vi "1.Create_Profile.vi"(8 "error out":errorcluster {"code" format="%.0x"}) -> (0 "error out":errorcluster {"code" format="%.0x"})   [LabVIEW 2021]
uses:
  test_type.ctl
  create profile state machine.ctl
panel:
  out "DCW":string[](array[string])
  out "output array":string[](array[string])
  out "IR":string[](array[string])
  out "Boolean":bool=TRUE
  out "Numeric":i32
  in  "Back Button":bool
  out "PROFILE TYPE 2":T1
  in  "String Indicator":string
  in  "Save Button":bool
  in  "Tab Control":enum32{"NA", "DCW", "ACW", "IR"}(tab)
  in  "DCW HI SET current value(mA)":sgl=11.0 min=0.001 max=11 format="%.3f"
  in  "DCW LO SET current value(mA)":sgl min=0 max=10.9 format="%.3f"
  in  "DCW Test Time(S)":sgl=0.5 min=0.5 max=999.9 format="%.1f"
  in  "DCW voltage(kV)":sgl=0.1 min=0.1 max=6.1 format="%.3f"
  in  "DCW Ramp Time":sgl=0.1 min=0.1 max=999.9 format="%.1f"
  in  "IR LO SET resistance value(M Ohm)":u16=2 min=1 max=9999
  in  "IR HI SET resistance value(M Ohm)":u16=9999 min=2 max=9999
  in  "IR Test Time(S)":sgl=1.0 min=1 max=999.9 format="%.1f"
  in  "Ramp Time":sgl=0.1 min=0.1 max=999.9 format="%.1f"
  in  "IR voltage(kV)":sgl=0.1 min=0.0499 max=1.0001 step=0.05 format="%.2f"
  in  "ACW Test Frequency(Hz)":u8(ring)=1 items=["50", "60"]
  in  "ACW Test Time(S)":sgl=0.5 min=0.5 max=999.9 format="%.1f"
  in  "ACW HI SET current value(mA)":sgl=42.0 min=0.001 max=42 format="%.3f"
  in  "ACW LO SET current value(mA)":sgl min=0 max=41.9 format="%.3f"
  in  "ACW voltage(kV)":sgl=0.1 min=0.1 max=5 format="%.3f"
  in  "ACW Ramp Time":sgl=0.1 min=0.1 max=999.9 format="%.1f"
  in  "PROFILE TYPE":T1
  # "CREATE PROFILE"
  # "PROFILE NAME"
  # "MODE"
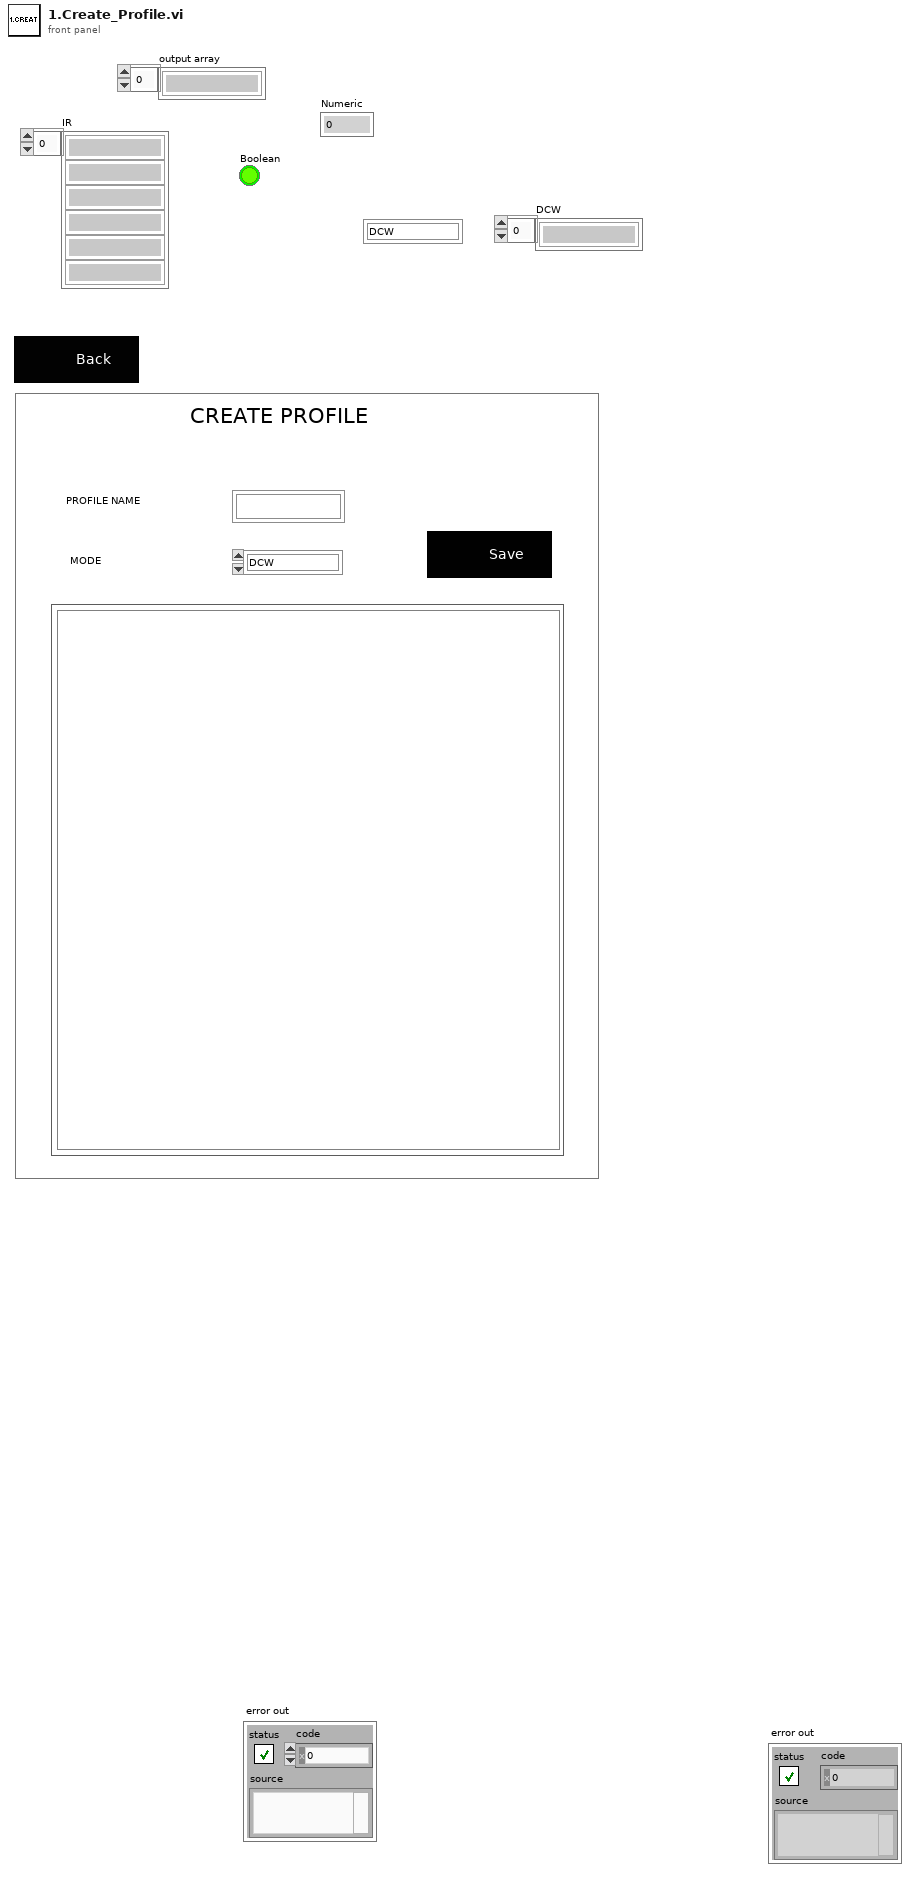
[diagram p1: front panel]
types:
  T1 = typedef "test_type.ctl" = enum16{"DCW", "ACW", "IR"}
  T2 = typedef "create profile state machine.ctl" = enum16{"Selection", "Compare name"}
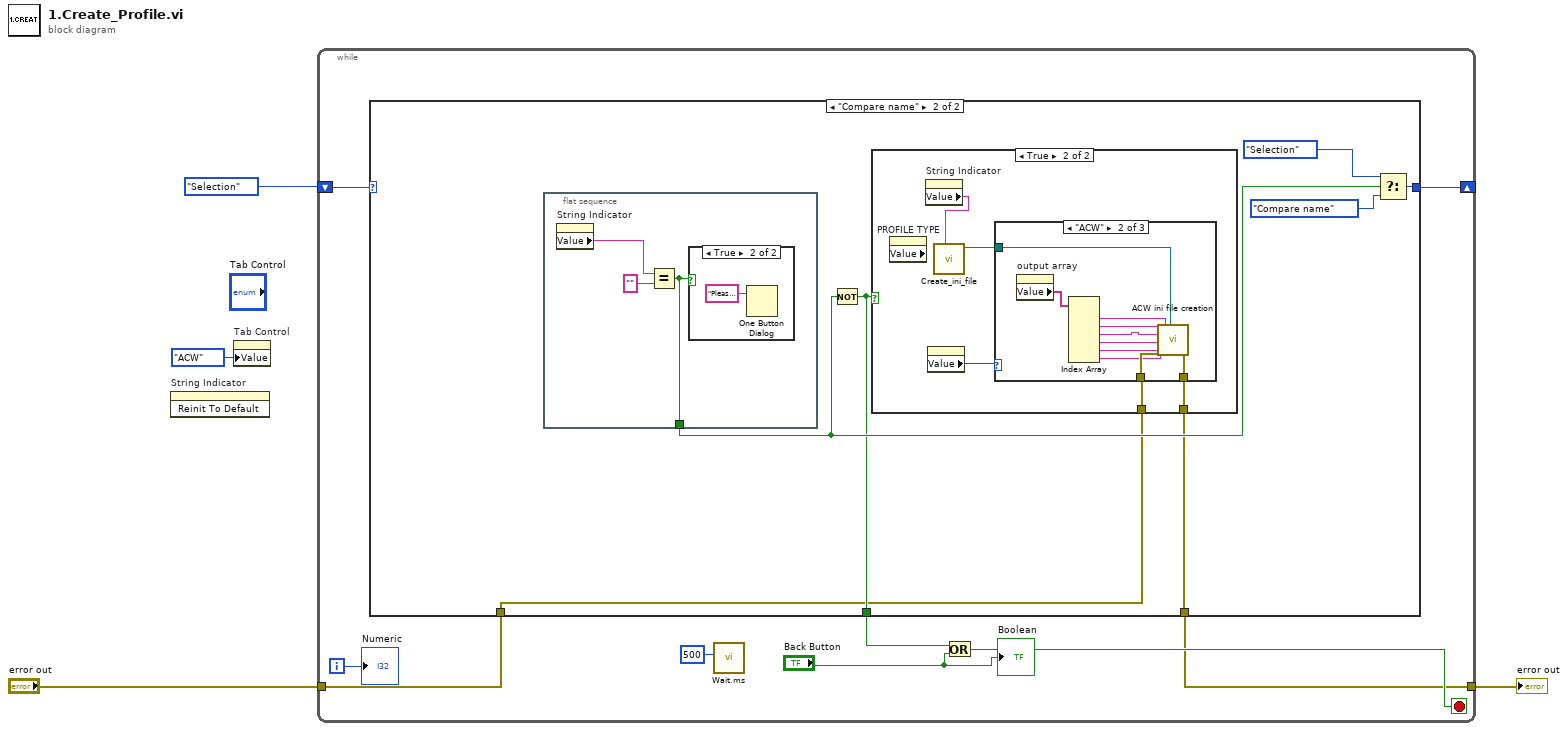
[diagram p0: block diagram]
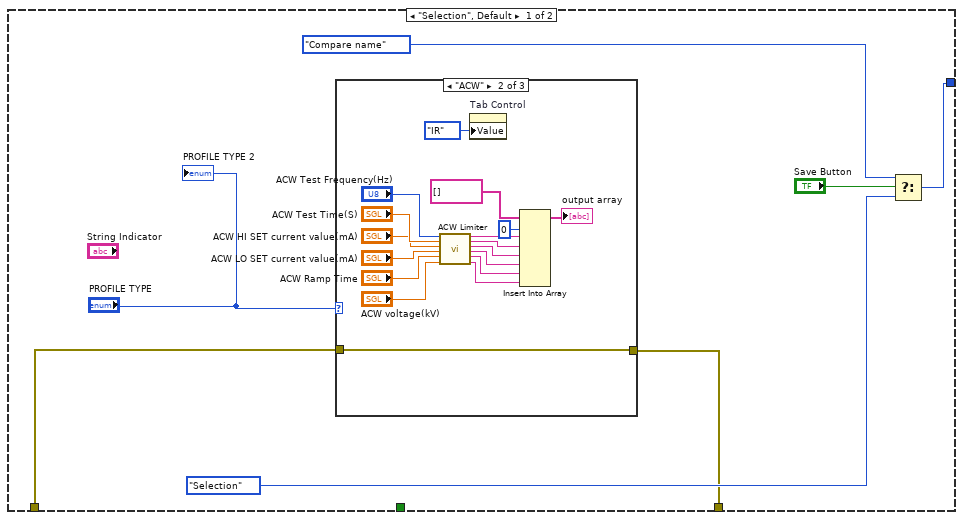
[diagram p2: hidden frame]
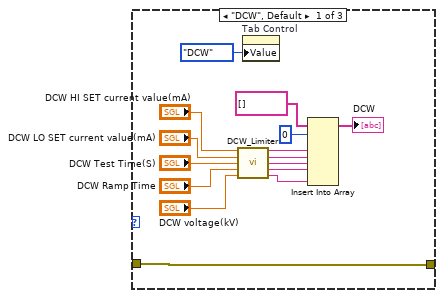
[diagram p3: hidden frame]
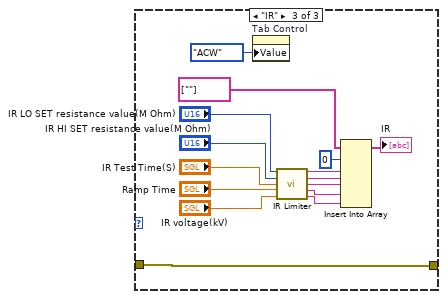
[diagram p4: hidden frame]
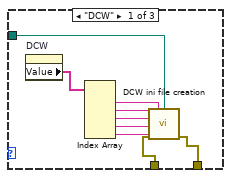
[diagram p6: hidden frame]
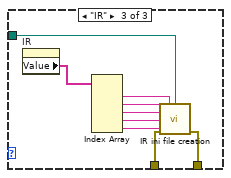
[diagram p7: hidden frame]
diagram:
  n1 = invoke on="String Indicator" class="Str" method="Reinit To Default"() -> ()  [unwired: 3 in, 3 out]
  n2 = property on="Tab Control" class="TabCtl (strict)"("Value"=enum32{"NA", "DCW", "ACW", "IR"}."ACW" ("Tab Control")) -> ()  [unwired: 2 in, 2 out]
  n3 = while {
    shift-right: [w12] -> _
    shift-left: create_profile_state_machine."Selection" -> [w13]
    tunnel: "error out" -> [w5]
    tunnel: [w6] -> w1
    i -> [w8]
    stop <- w9 stop-if-true
    n4 = case shown="\"Compare name\"" w13 {
      tunnel: [w20 w73] -> w12
      tunnel: w5 -> [w16 w68]
      tunnel: [_ w70] -> w10
      tunnel: [w14 w69] -> w6
      frame "Selection", Default {
        n5 = case shown="\"ACW\"" "PROFILE TYPE" {
          tunnel: w16 -> [w34 w51 w66]
          tunnel: [w34 w51 w66] -> w14
          frame "DCW", Default {
            n6 = call "DCW_Limiter.vi"("DCW HI SET current value(mA)"="DCW HI SET current value(mA)", "DCW LO SET current value(mA)"="DCW LO SET current value(mA)", "DCW Test Time(S)"="DCW Test Time(S)", "Ramp Time"="DCW Ramp Time", "DCW voltage(kV)"="DCW voltage(kV)") -> ("DCW voltage(kV)"=w33:string, "Ramp Time"=w32:string, "DCW LO SET current value(mA)"=w31:string, "DCW HI SET current value(mA)"=w30:string, "DCW Test Time(S)"=w29:string)  [unwired: 6 in]
            n7 = property on="Tab Control" class="TabCtl (strict)"("Value"=enum32{"NA", "DCW", "ACW", "IR"}."DCW" ("Tab Control")) -> ()  [unwired: 2 in, 2 out]
            n8 = Insert Into Array(array=string[] [], index=0, new element #1=w33, new element #2=w32, new element #3=w31, new element #4=w30, new element #5=w29) -> (→"DCW":string[])
          }
          frame "ACW" {
            n9 = call "ACW Limiter.vi"("ACW Test Frequency(Hz)"="ACW Test Frequency(Hz)", "ACW Test Time(S)"="ACW Test Time(S)", "ACW HI SET current value(mA)"="ACW HI SET current value(mA)", "ACW LO SET current value(mA)"="ACW LO SET current value(mA)", "Ramp Time"="ACW Ramp Time", "ACW voltage(kV)"="ACW voltage(kV)") -> ("ACW voltage(kV)"=w50:string, "Ramp Time"=w49:string, "ACW LO SET current value(mA)"=w48:string, "ACW HI SET current value(mA)"=w47:string, "ACW Test Time(S)"=w46:string, "ACW Test Frequency(Hz)"=w45:string)  [unwired: 8 in]
            n10 = property on="Tab Control" class="TabCtl (strict)"("Value"=enum32{"NA", "DCW", "ACW", "IR"}."IR" ("Tab Control")) -> ()  [unwired: 2 in, 2 out]
            n11 = Insert Into Array(array=string[] [], index=0, new element #1=w50, new element #2=w49, new element #3=w48, new element #4=w47, new element #5=w46, new element #6=w45) -> (→"output array":string[])
          }
          frame "IR" {
            n12 = property on="Tab Control" class="TabCtl (strict)"("Value"=enum32{"NA", "DCW", "ACW", "IR"}."ACW" ("Tab Control")) -> ()  [unwired: 2 in, 2 out]
            n13 = call "IR Limiter.vi"("IR LO SET resistance value(M£[)"="IR LO SET resistance value(M Ohm)", "IR HI SET resistance value(M£[)"="IR HI SET resistance value(M Ohm)", "IR Test Time(S)"="IR Test Time(S)", "Ramp Time"="Ramp Time", "IR voltage(kV)"="IR voltage(kV)") -> ("IR voltage(kV)"=w65:string, "IR Test Time(S)"=w64:string, "IR LO SET"=w63:string, "IR HI SET"=w62:string, "Ramp Time"=w61:string)  [unwired: 6 in]
            n14 = Insert Into Array(array=string[] [""], index=0, new element #1=w65, new element #2=w64, new element #3=w63, new element #4=w62, new element #5=w61) -> (→"IR":string[])
          }
        }
        n15 = Select(t=create_profile_state_machine."Compare name", s="Save Button", f=create_profile_state_machine."Selection") -> (s? t:f=w20:T2)
        "PROFILE TYPE 2" <- "PROFILE TYPE"
      }
      frame "Compare name" {
        n16 = flat-sequence {
          tunnel: [w110] -> w71
          frame #0 {
            n17 = property on="String Indicator" class="Str"() -> ("Value"=w109:string)  [unwired: 2 in, 2 out]
            n18 = Equal?(x=w109, y="") -> (x = y?=w110:bool)
            n19 = case shown="True" w110 {
              frame False {
              }
              frame True {
                n20 = One Button Dialog(message="Please enter the Profile Name") -> ()  [unwired: 1 in, 1 out]
              }
            }
          }
        }
        n21 = Not(x=w71) -> (.not. x?=w70:bool)
        n22 = case shown="True" w70 {
          tunnel: [w75 w77] -> w69
          tunnel: w68 -> [w75 w76]
          frame False {
          }
          frame True {
            n23 = property on="PROFILE TYPE" class="Enum (strict)" props=["Value"]() -> ()  [unwired: 2 in, 3 out]
            n24 = property on="String Indicator" class="Str"() -> ("Value"=w79:string)  [unwired: 2 in, 2 out]
            n25 = property on="PROFILE TYPE 2" class="Enum (strict)"() -> ("Value"=w78:T1)  [unwired: 2 in, 2 out]
            n26 = call "Create_ini_file.vi"("Name"=w79) -> ("path"=w80:path)  [unwired: 9 in, 1 out]
            n27 = case shown="\"ACW\"" w78 {
              tunnel: w80 -> [w89 w95 w108]
              tunnel: [w88 w99 w107] -> w77
              tunnel: w76 -> [w87 w98 w106]
              frame "DCW" {
                n28 = property on="DCW" class="Arr (strict)"() -> ("Value"=w86:string[])  [unwired: 2 in, 2 out]
                n29 = Index Array(array=w86) -> (element #1=w85:string, element #2=w84:string, element #3=w83:string, element #4=w82:string, element #5=w81:string)  [unwired: 5 in]
                n30 = call "DCW ini file creation.vi"("Ramp Time"=w84, "DCW voltage(kV)"=w85, "configuration file path"=w89, "DCW LO SET current value(mA)"=w83, "DCW HI SET current value(mA)"=w82, "DCW Test Time(S)"=w81, "error in (no error) 2"=w87) -> ("error in (no error) 3"=w88:errorcluster)  [unwired: 8 in]
              }
              frame "ACW" {
                n31 = property on="output array" class="Arr (strict)"() -> ("Value"=w97:string[])  [unwired: 2 in, 2 out]
                n32 = Index Array(array=w97) -> (element #1=w96:string, element #2=w94:string, element #3=w93:string, element #4=w92:string, element #5=w90:string, element #6=w91:string)  [unwired: 6 in]
                n33 = call "ACW ini file creation.vi"("Ramp Time"=w94, "ACW LO SET current value(mA)"=w93, "ACW HI SET current value(mA)"=w92, "ACW Test Time(S)"=w90, "ACW Test Frequency(Hz)"=w91, "error in (no error) 2"=w98, "ACW voltage(kV)"=w96, "configuration file path"=w95) -> ("error in (no error) 3"=w99:errorcluster)  [unwired: 11 in]
              }
              frame "IR" {
                n34 = property on="IR" class="Arr (strict)"() -> ("Value"=w105:string[])  [unwired: 2 in, 2 out]
                n35 = Index Array(array=w105) -> (element #1=w104:string, element #2=w103:string, element #3=w102:string, element #4=w101:string, element #5=w100:string)  [unwired: 5 in]
                n36 = call "IR ini file creation.vi"("IR Test Time(S)"=w103, "IR voltage(kV)"=w104, "configuration file path"=w108, "IR LO SET"=w102, "IR HI SET"=w101, "Ramp Time"=w100, "error in (no error) 2"=w106) -> ("error in (no error) 3"=w107:errorcluster)  [unwired: 8 in]
              }
            }
          }
        }
        n37 = Select(t=create_profile_state_machine."Selection", s=w71, f=create_profile_state_machine."Compare name") -> (s? t:f=w73:T2)
      }
    }
    n38 = call "Wait.ms.vi"("milliseconds to wait"=u32 500) -> ()  [unwired: 10 in, 1 out]
    n39 = Or(x=w10, y="Back Button") -> (x .or. y?=w9:bool)
    "Numeric" <- w8
    "Boolean" <- "Back Button"
  }
  "error out" <- w1
